vi "Filters.vi"() -> ()   [LabVIEW 2026]
panel:
  out "Clean Composite Signal":waveform(dbl)(graph)
  out "Original  Noisy Signal":waveform(dbl)(graph)
  in  "Signal Parameters":T1
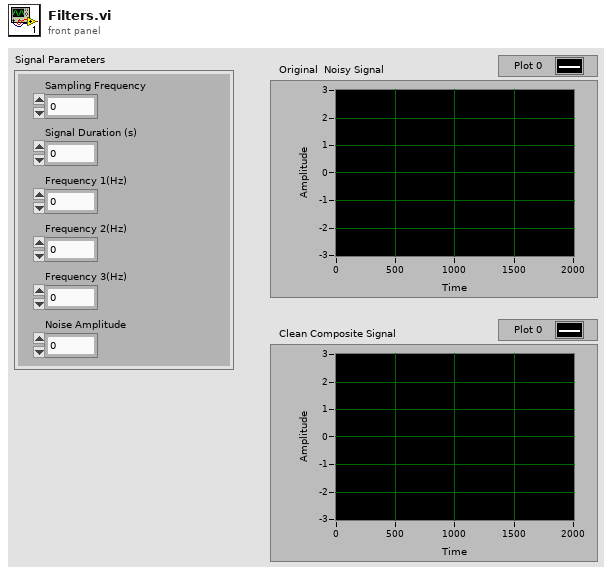
[diagram p1: front panel]
types:
  T1 = cluster{"Sampling Frequency":dbl, "Signal Duration (s)":dbl, "Frequency 1(Hz)":dbl, "Frequency 2(Hz)":dbl, "Frequency 3(Hz)":dbl, "Noise Amplitude":dbl}
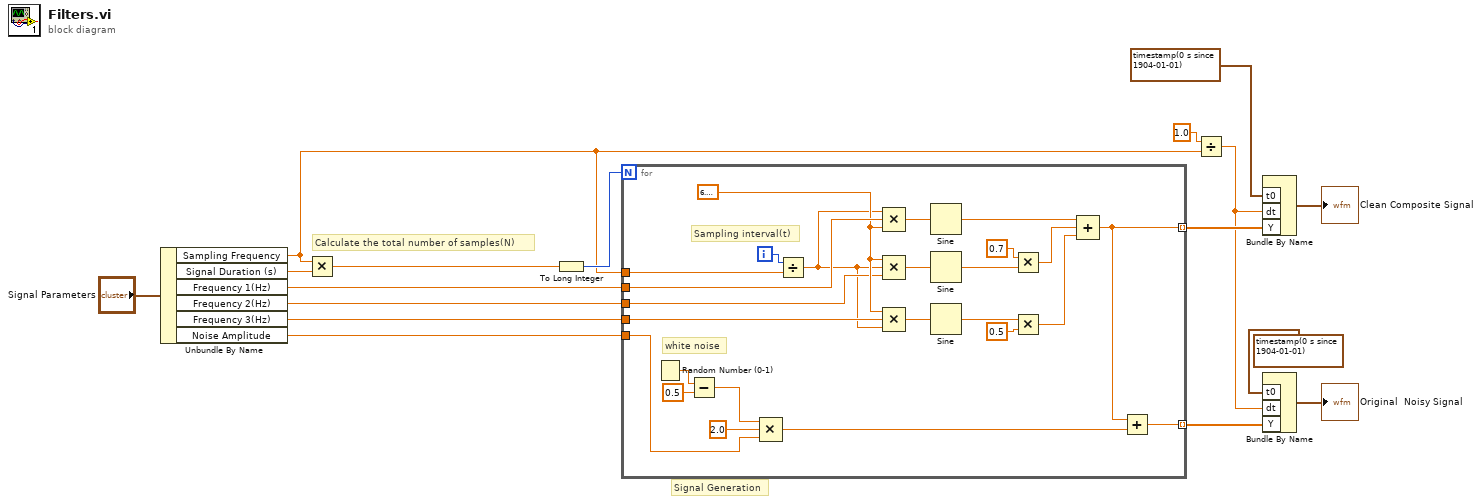
[diagram p0: block diagram]
diagram:
  # "Signal Generation"
  # "Calculate the total number of samples(N)"
  n1 = Unbundle By Name("Signal Parameters") -> ("Sampling Frequency"=w7:dbl, "Signal Duration (s)"=w16:dbl, "Frequency 1(Hz)"=w15:dbl, "Frequency 2(Hz)"=w14:dbl, "Frequency 3(Hz)"=w13:dbl, "Noise Amplitude"=w12:dbl)
  n2 = Multiply(x=w7, y=w16) -> (x*y=w11:dbl)
  n3 = To Long Integer(number=w11) -> (32bit integer=w10:i32)
  n4 = for {
    N: w10 -> [_]
    tunnel: w7 -> [w41]
    tunnel: w15 -> [w40]
    tunnel: w14 -> [w34]
    tunnel: w13 -> [w33]
    tunnel: w12 -> [w21]
    tunnel: [w19] -> w4 mode=indexing
    tunnel: [w18] -> w9 mode=indexing
    i -> [w42]
    w35 = 6.283185307179586
    # "white noise"
    # "Sampling interval(t)"
    n5 = Random Number (0-1)() -> (number: 0 to 1=w25:dbl)
    n6 = Subtract(x=w25, y=0.5) -> (x-y=w23:dbl)
    n7 = Compound Arithmetic op=MULTIPLY(w23, 2.0 ("y"), w21) -> (w20:dbl)
    n8 = Divide(x=w42, y=w41) -> (x/y=w32:dbl)
    n9 = Compound Arithmetic op=MULTIPLY(w32, w40, w35) -> (w39:dbl)
    n10 = Compound Arithmetic op=MULTIPLY(w35, w32, w34) -> (w36:dbl)
    n11 = Compound Arithmetic op=MULTIPLY(w35, w33, w32) -> (w31:dbl)
    n12 = Sine(x=w39) -> (sin(x)=w28:dbl)
    n13 = Sine(x=w36) -> (sin(x)=w38:dbl)
    n14 = Sine(x=w31) -> (sin(x)=w30:dbl)
    n15 = Multiply(x=0.7, y=w38) -> (x*y=w27:dbl)
    n16 = Multiply(x=w30, y=0.5) -> (x*y=w26:dbl)
    n17 = Compound Arithmetic op=ADD(w28, w27, w26) -> (w18:dbl)
    n18 = Add(x=w18, y=w20) -> (x+y=w19:dbl)
  }
  n19 = Divide(x=1.0, y=w7) -> (x/y=w3:dbl)
  n20 = Bundle By Name("t0"=timestamp(0 s since 1904-01-01), "dt"=w3, "Y"=w9) -> (→"Clean Composite Signal":waveform(dbl))  [unwired: 1 in]
  n21 = Bundle By Name("t0"=timestamp(0 s since 1904-01-01), "dt"=w3, "Y"=w4) -> (→"Original  Noisy Signal":waveform(dbl))  [unwired: 1 in]
